vi "Tell If Stopped.vi"(4 "Priority":bool, 9 "Msg":refnum<class "Msg.lvclass">, 10 "Transport":refnum<class "Transport.lvclass">) -> (0 "Error out":errorcluster)   [LabVIEW 2020, in "jettl.lvlib"]
uses:
  jettl.lvlib
  Msg/Msg.lvclass
  Transport/Transport.lvclass
  Stopped jettl Msg/Stopped/Init Msg Default.vi
  Stopped jettl Msg/Stopped Msg/Init Msg Default.vi
  Stopped jettl Msg/Stopped Msg/Stopped Msg/Init Msg Default.vi
  Stopped jettl Msg/Stopped Msg/Stopped Msg/Stopped Msg.lvclass
  C:/git/jettl/src/jettl/jettl/Msg/Msg.lvclass
  Stopped jettl Msg/Stopped/Stopped.lvlib
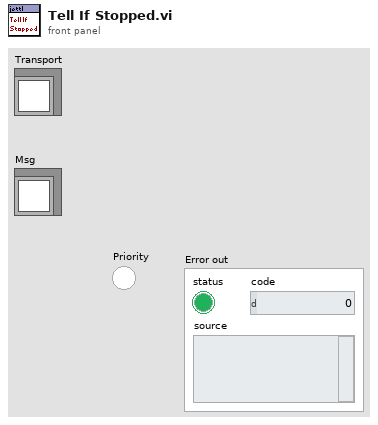
[diagram p1: front panel]
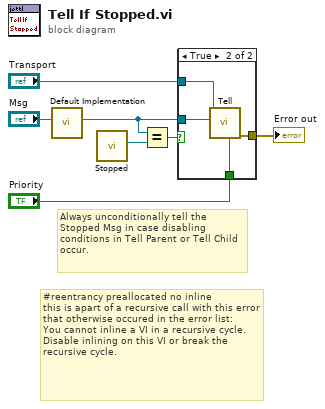
[diagram p0: block diagram]
diagram:
  # "#reentrancy preallocated no inline\nthis is apart of a recursive call with this error that otherwise occured in the error list:\nYou cannot inline a VI in a recursive cycle. Disable inlining on this VI or break the recursive cycle."
  # "Always unconditionally tell the Stopped Msg in case disabling conditions in Tell Parent or Tell Child occur."
  n1 = call "Default Implementation.vi"("Implementation"="Msg") -> ("Default Implementation"=w1:refnum<class "Msg.lvclass">)  [unwired: 10 in]
  n2 = call-poly "Stopped.vi"() -> ("Msg"=w3:refnum<class "Msg.lvclass">)  [unwired: 11 in]
  n3 = Equal?(x=w1, y=w3) -> (x = y?=w7:bool)
  n4 = case shown="True" w7 {
    tunnel: "Transport" -> [_ w11]
    tunnel: "Priority" -> [_ w10]
    tunnel: [_ w9] -> w6
    tunnel: w1 -> [_ w8]
    frame False {
    }
    frame True {
      n5 = call-dynamic "Tell.vi"("Priority"=w10, "Msg"=w8, "Transport in"=w11) -> ("Error out"=w9:errorcluster)  [unwired: 8 in]
    }
  }
  "Error out" <- w6
